vi "EPC300X Initialize.vi"(0 "VISA resource name":refnum<visa-resource-name>="ASRL1::INSTR", 1 "Unit Address (1)":u8=1, 5 "ID Query? (T: Yes)":bool=TRUE, 7 "Serial Configuration":T1={"Baud Rate (9600)"=9600, "Parity (0: None)"=0, "Break Length (0)"=20} {"Break Length (0)" items=["0"=10, "1.5"=15, "2.0"=20]; "Parity (0: None)" items=["None", "Odd", "Even"]; "Baud Rate (9600)" items=["300"=300, "600"=600, "1200"=1200, "2400"=2400, "4800"=4800, "9600"=9600, "19200"=19200]}, 11 "error in (no error)":errorcluster) -> (4 "VISA resource name out":refnum<visa-resource-name>, 15 "error out":errorcluster {"code" format="%x"})   [LabVIEW 2022 SP3]
doc: "This VI passes the addressing information in the instrument decriptor to the Instr Open VI and returns the instrument ID. You must run this VI before using any of the instrument driver VIs for this instrument.\n\nNotes:\n\n(1) This instrument driver supports serial communication. If problems are encountered when using serial communication, it is recommended to try using baud rates less than 19,200 and hardware handshaking. \n\n(2) If you do wish to use the serial interface, set the serial settings on the instrument to be the same as the serial settings on the block diagram and in Measurement & Automation Explorer."
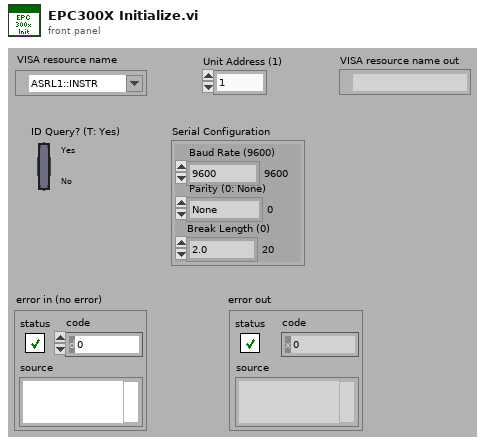
[diagram p1: front panel]
types:
  T1 = cluster{"Baud Rate (9600)":u32, "Parity (0: None)":u16, "Break Length (0)":u16}
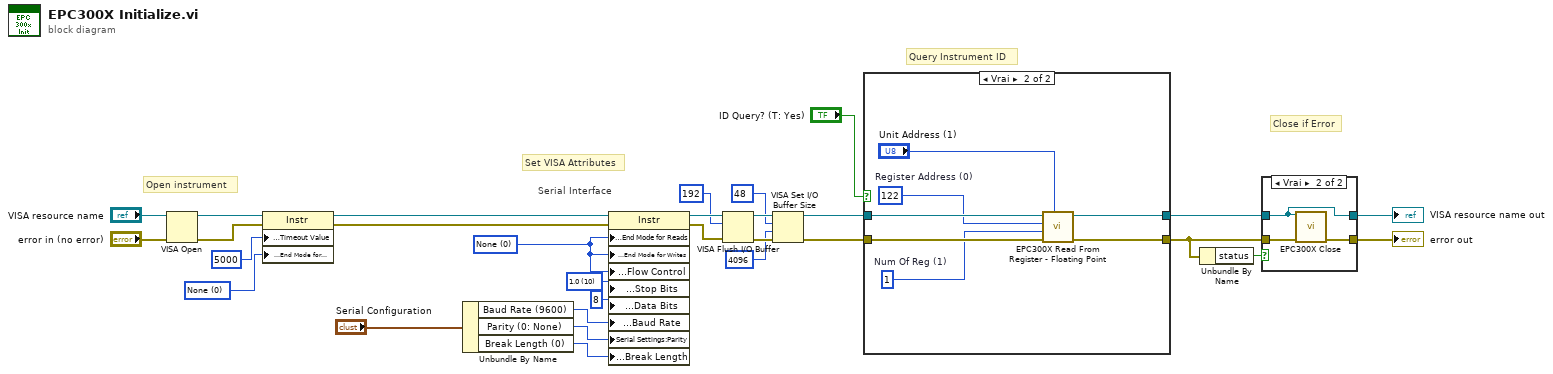
[diagram p0: block diagram]
diagram:
  w5 = u16 10 items=["1.0"=10, "1.5"=15, "2.0"=20] ("Serial Settings:Serial Stop Bits")
  w6 = u16 0 items=["None", "LastBit", "TermChar"] ("Serial Settings:Serial End Mode for Reads")
  w19 = u16 0 items=["None", "LastBit", "TermChar"] ("Serial Settings:Serial End Mode for Reads")
  # "Serial Interface"
  # "Set VISA Attributes"
  # "Close if Error"
  # "Query Instrument ID"
  # "Open instrument"
  n1 = VISA Open(error in (no error)="error in (no error)", VISA resource name="VISA resource name") -> (VISA resource name=w18:refnum<visa-resource-name>, error out=w17:errorcluster)  [unwired: 3 in]
  n2 = property class="Instr"(reference=w18, error in=w17, "General Settings:Timeout Value"=u32 5000, "Serial Settings:End Mode for Reads"=w19) -> (reference out=w22:refnum<visa-resource-name>, error out=w21:errorcluster)
  n3 = Unbundle By Name("Serial Configuration") -> ("Baud Rate (9600)"=w3:u32, "Parity (0: None)"=w2:u16, "Break Length (0)"=w1:u16)
  n4 = property class="Instr"(reference=w22, error in=w21, "Serial Settings:End Mode for Reads"=w6, "Serial Settings:End Mode for Writes"=w6, "Serial Settings:Flow Control"=w6, "Serial Settings:Stop Bits"=w5, "Serial Settings:Data Bits"=u16 8 ("Serial Settings:Serial Data Bits"), "Serial Settings:Baud Rate"=w3, "Serial Settings:Parity"=w2, "Serial Settings:Break Length"=w1) -> (reference out=w11:refnum<visa-resource-name>, error out=w13:errorcluster)
  n5 = VISA Flush I/O Buffer(VISA resource name=w11, mask (16)=u16 192, error in (no error)=w13) -> (VISA resource name out=w14:refnum<visa-resource-name>, error out=w12:errorcluster)
  n6 = VISA Set I/O Buffer Size(VISA resource name=w14, mask (16)=u16 48, size (4096)=u32 4096 ("size (0)"), error in (no error)=w12) -> (VISA resource name out=w24:refnum<visa-resource-name>, error out=w23:errorcluster)
  n7 = case shown="Vrai" "ID Query? (T: Yes)" {
    tunnel: [w32 w33] -> w15
    tunnel: [w31 w38] -> w16
    tunnel: w24 -> [w31 w39]
    tunnel: w23 -> [w32 w37]
    frame False {
    }
    frame True {
      w36 = u16 1  # Num Of Reg (1)
      w34 = u16 122  # Register Address (0)
      n8 = call "EPC300X Read From Register - Floating Point.vi"("Unit Address (1)"="Unit Address (1)", "error in (no error)"=w37, "Num Of Reg (1)"=w36, "Register Address (0)"=w34, "VISA session"=w39) -> ("error out"=w33:errorcluster, "dup VISA session"=w38:refnum<visa-resource-name>)  [unwired: 1 in, 4 out]
    }
  }
  n9 = Unbundle By Name(w15) -> ("status"=w20:bool)
  n10 = case shown="Vrai" w20 {
    tunnel: w16 -> [w41 w43]
    tunnel: [w41 w43] -> w29
    tunnel: [w40 w44] -> w28
    tunnel: w15 -> [w40 w42]
    frame False {
    }
    frame True {
      n11 = call "EPC300X Close.vi"("VISA resource name"=w43, "error in (no error)"=w42) -> ("error out"=w44:errorcluster)  [unwired: 13 in]
    }
  }
  "VISA resource name out" <- w29
  "error out" <- w28
